vi "Remove Language from translations.vi"(8 "Unicode Index":i32, 9 "ANSI Index":i32, 11 "Translastions in":map{string, T1}(c390)) -> (3 "Translastions out":map{string, T1}(c390))   [LabVIEW 2019, in "Language Editor.lvlib"]
doc: "- - -\nCopyright (c) 2026, Merecs Engineering GmbH"
uses:
  Language Editor.lvlib
  type defs/Cluster Translations.ctl
  Language Selection/TypeDefs/Cluster PropertyTranslation.ctl
  Language Selection/TypeDefs/Enum Property Type.ctl
  Language Selection/Language Selection.lvlib
panel:
  # "Connector Pane"
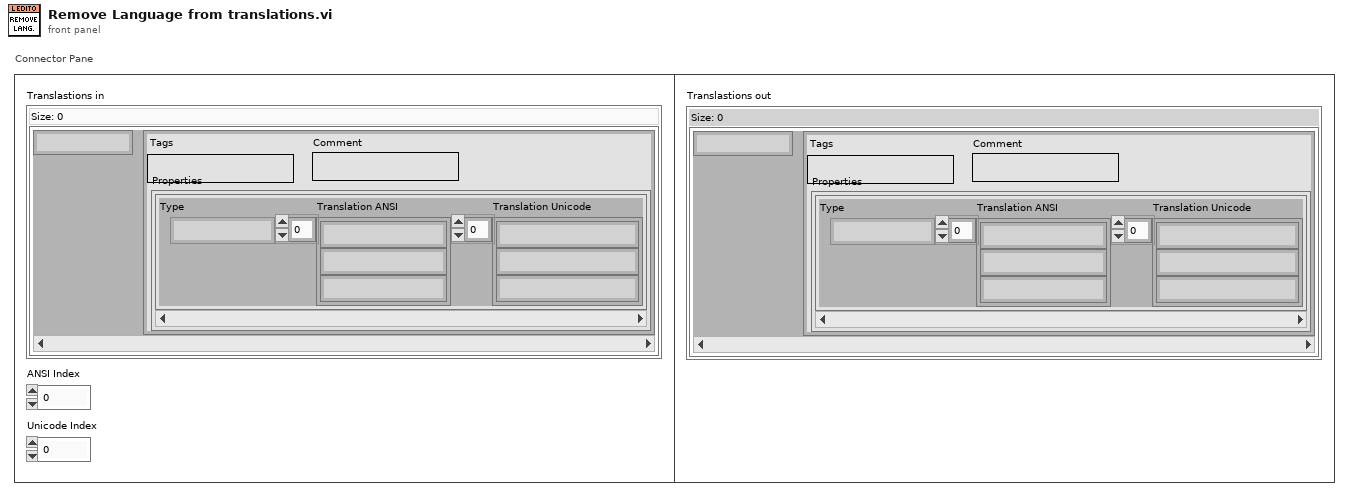
[diagram p1: front panel]
types:
  T1 = typedef "Language Editor.lvlib/Cluster Translations.ctl" = cluster{"Tags":string, "Comment":string, "Properties":T2[]}
  T2 = typedef "Language Selection.lvlib/Cluster PropertyTranslation.ctl" = cluster{"Type":T3, "Translation ANSI":string[], "Translation Unicode":string[]}
  T3 = typedef "Language Selection.lvlib/Enum Property Type.ctl" = enum16{"NA", "Caption", "String Value", "Boolean Text", "Ring Strings", "1D Array Elements", "2D Array Elements", "(MC)Listbox Header", "(MC)Listbox Items", "Tab Pages Names", "X & Y GraphChart", "Plot Names", "Table Headers", "Table Items", "TipStrip", "Combobox Strings", "Cursor Name", "Tree Col Headers"}
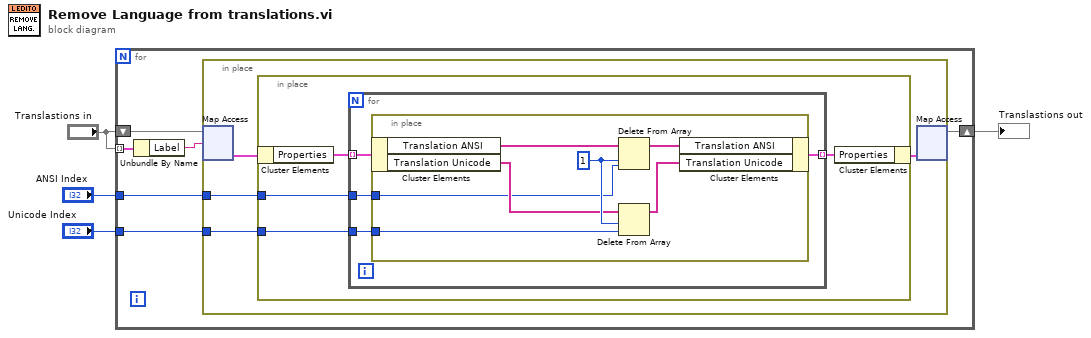
[diagram p0: block diagram]
diagram:
  n1 = for {
    shift-right: [w9] -> w3
    shift-left: "Translastions in" -> [w10]
    tunnel: "Translastions in" -> [w8] mode=indexing
    tunnel: "Unicode Index" -> [w6]
    tunnel: "ANSI Index" -> [w5]
    n2 = Unbundle By Name(w8) -> ("Label"=w7:string)
    n3 = in-place {
      in-place-border: w6 -> [w12]
      in-place-border: w5 -> [w11]
      n4 = in-place-map #1(w10, w7) -> (w14:T1)  [unwired: 1 in, 1 out]
      n5 = in-place {
        in-place-border: w12 -> [w16]
        in-place-border: w11 -> [w15]
        n6 = in-place-cluster #2(w14) -> ("Properties"=w18:T2[])
        n7 = for {
          tunnel: w18 -> [w21] mode=indexing
          tunnel: [w22] -> w17 mode=indexing
          tunnel: w16 -> [w20]
          tunnel: w15 -> [w19]
          n8 = in-place {
            in-place-border: w20 -> [w25]
            in-place-border: w19 -> [w23]
            w26 = 1 ("length")
            n9 = in-place-cluster #3(w21) -> ("Translation ANSI"=w29:string[], "Translation Unicode"=w24:string[])
            n10 = Delete From Array(array=w29, length=w26, index=w23) -> (array with subset deleted=w28:string[])  [unwired: 1 out]
            n11 = Delete From Array(array=w24, length=w26, index=w25) -> (array with subset deleted=w27:string[])  [unwired: 1 out]
            n12 = in-place-cluster #3("Translation ANSI"=w28, "Translation Unicode"=w27) -> (w22:T2)
          }
        }
        n13 = in-place-cluster #2("Properties"=w17) -> (w13:T1)
      }
      n14 = in-place-map #1(w13) -> (w9:map{string, T1})  [unwired: 1 in, 2 out]
    }
  }
  "Translastions out" <- w3
